vi "Modbus Master.vi"() -> ()   [LabVIEW 2021]
uses:
  TypeDefs/Tester Object.ctl
  TypeDefs/UIControlReferences.ctl
  TypeDefs/Devices Cluster.ctl
  Modbus/Modbus Cluster.ctl
  <vilib>/NI/Modbus Library/API/Master/Modbus Master.lvclass
  Modbus/Modbus Address Cluster.ctl
  <vilib>/NI/Modbus Library/API/Slave/Modbus Slave.lvclass
  DAQ/DAQNav/DAQNav Cluster.ctl
  DAQ/DAQNav/Analog Cluster.ctl
panel:
  out "Register Values":dbl[](array[numeric])
  in  "stop":bool
  out "error out":errorcluster
  out "Motor Speed":dbl
  out "Temperature":dbl
  out "Positioning":dbl
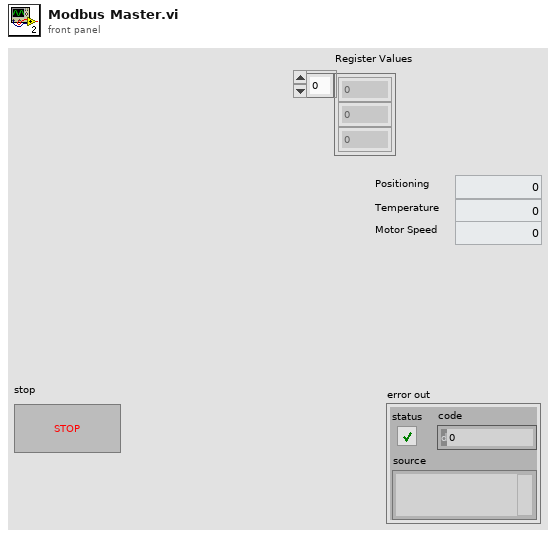
[diagram p1: front panel]
types:
  T1 = typedef "Tester Object.ctl" = cluster{"Program Properties":cluster{"Application Path":path}, "Control Refnum":T2, "Devices":T3}
  T2 = typedef "UIControlReferences.ctl" = cluster{"Tree Refnum ":refnum<vi>, "Graph1 Refnum":refnum<vi>, "Graph2 Refnum":refnum<vi>, "Temperature Refnum":refnum<vi>, "Sensor Str Refnum":refnum<vi>, "Motor Speed Refnum":refnum<vi>, "Equipment Connected Refnum":refnum<vi>, "Calibrated Refnum":refnum<vi>, "Positioning Refnum":refnum<vi>, "Servo On Refnum":refnum<vi>, "seqPauseButton":refnum<vi>, "seqStartButton":refnum<vi>, "seqStopButton":refnum<vi>}
  T3 = typedef "Devices Cluster.ctl" = cluster{"Modbus":T4, "TCP/IP":cluster{"connection ID":refnum<k5>, "Address":string}, "DAQ Device":T6}
  T4 = typedef "Modbus Cluster.ctl" = cluster{"Modbus master instance":refnum<class "Modbus Master.lvclass">, "MB Holding Register":T5[], "MB Coils":T5[], "TCP slave instance":refnum<class "Modbus Slave.lvclass">}
  T5 = typedef "Modbus Address Cluster.ctl" = cluster{"Session":string, "Device Type":string, "Memory Block":string, "Function":string, "Address":u16}
  T6 = typedef "DAQNav Cluster.ctl" = cluster{"AI task out":i32, "AI Found?":bool, "AO task out":i32, "AO Found?":bool, "Analog Input List":T7[], "Analog Out List":T7[]}
  T7 = typedef "Analog Cluster.ctl" = cluster{"Name":string, "Device Type":string, "Channel":i32}
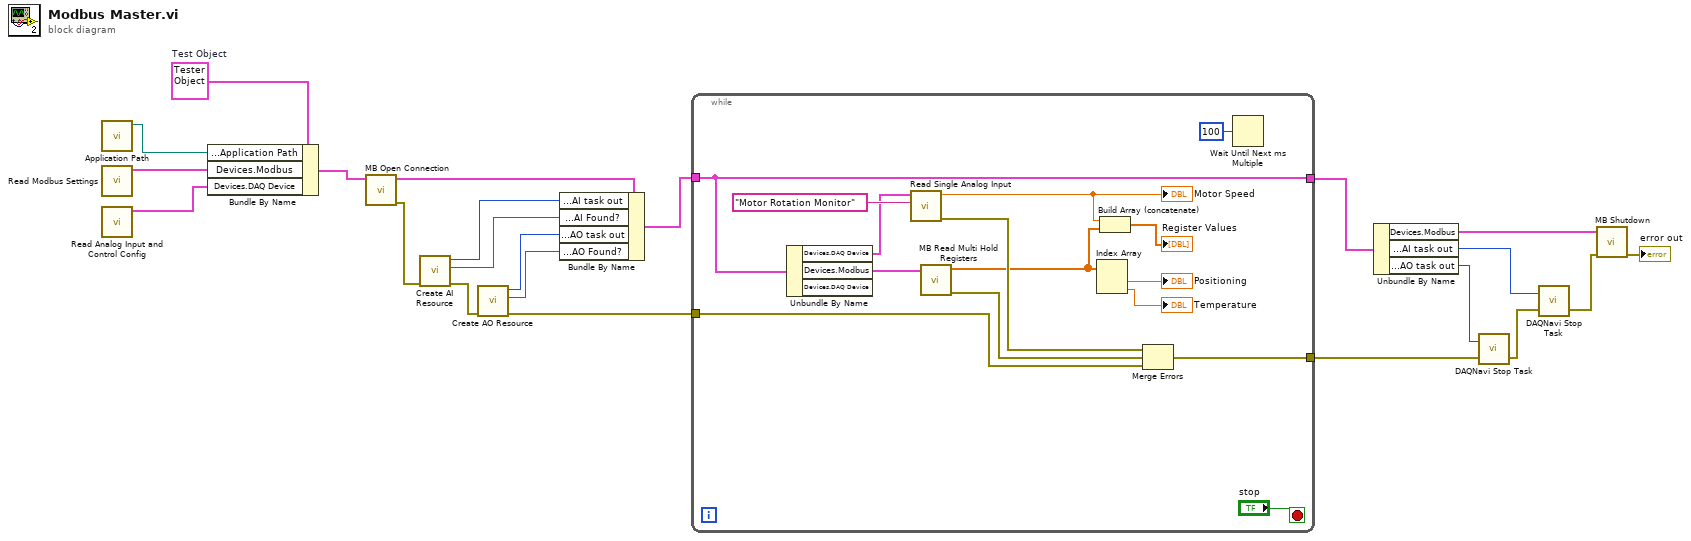
[diagram p0: block diagram]
diagram:
  w22 = T1 {"Program Properties"={"Application Path"=path ""}, "Control Refnum"={"Tree Refnum "=refnum, "Graph1 Refnum"=refnum, "Graph2 Refnum"=refnum, "Temperature Refnum"=refnum, "Sensor Str Refnum"=refnum, "Motor Speed Refnum"=refnum, "Equipment Connected Refnum"=refnum, "Calibrated Refnum"=refnum, "Positioning Refnum"=refnum, "Servo On Refnum"=refnum, "seqPauseButton"=refnum, "seqStartButton"=refnum, "seqStopButton"=refnum}, "Devices"={"Modbus"={"Modbus master instance"=refnum, "MB Holding Register"=[], "MB Coils"=[], "TCP slave instance"=refnum}, "TCP/IP"={"connection ID"=refnum, "Address"=""}, "DAQ Device"={"AI task out"=0, "AI Found?"=FALSE, "AO task out"=0, "AO Found?"=FALSE, "Analog Input List"=[], "Analog Out List"=[]}}}  # Test Object
  n1 = call "Application Path.vi"() -> ("appended path"=w1:path)  [unwired: 11 in]
  n2 = call "Read Modbus Settings.vi"() -> ("Devices.Modbus"=w21:T4)  [unwired: 11 in]
  n3 = call "Read Analog Input and Control Config.vi"() -> ("daq cluster"=w20:T6)  [unwired: 11 in]
  n4 = Bundle By Name(cluster=w22, "Program Properties.Application Path"=w1, "Devices.Modbus"=w21, "Devices.DAQ Device"=w20) -> (w19:T1)
  n5 = call "MB Open Connection.vi"("Test Object in"=w19) -> ("error out"=w3:errorcluster, "Test Object out"=w18:T1)  [unwired: 9 in]
  n6 = call "Create AI Resource.vi"("error in (no error)"=w3) -> ("error out"=w2:errorcluster, "found?"=w16:bool, "task out"=w17:i32)  [unwired: 8 in]
  n7 = call "Create AO Resource.vi"("error in (no error)"=w2) -> ("error out"=w4:errorcluster, "found?"=w14:bool, "task out"=w15:i32)  [unwired: 8 in]
  n8 = Bundle By Name(cluster=w18, "Devices.DAQ Device.AI task out"=w17, "Devices.DAQ Device.AI Found?"=w16, "Devices.DAQ Device.AO task out"=w15, "Devices.DAQ Device.AO Found?"=w14) -> (w13:T1)
  n9 = while {
    tunnel: w13 -> [w34]
    tunnel: [w34] -> w9
    tunnel: [w33] -> w8
    tunnel: w4 -> [w32]
    stop <- "stop" stop-if-true
    n10 = Unbundle By Name(w34) -> ("Devices.DAQ Device"=w23:T6, "Devices.Modbus"=w37:T4)  [unwired: 1 out]
    n11 = call "Read Single Analog Input.vi"("Parameter Name"="Motor Rotation Monitor", "Devices.DAQ Device"=w23) -> ("error out"=w28:errorcluster, "data"=w26:dbl)  [unwired: 7 in, 1 out]
    "Motor Speed" <- w26
    n12 = call "MB Read Multi Hold Registers.vi"("Devices.Modbus"=w37) -> ("error out"=w27:errorcluster, "Register Values"=w25:dbl[])  [unwired: 9 in]
    n13 = Index Array(array=w25) -> (element #1=→"Positioning":dbl, element #2=→"Temperature":dbl)  [unwired: 2 in]
    n14 = Build Array (concatenate)(w26, w25) -> (→"Register Values":dbl[])
    n15 = Merge Errors(w28, w27, w32) -> (w33:errorcluster)
    n16 = Wait Until Next ms Multiple(millisecond multiple=u32 100) -> ()  [unwired: 1 out]
  }
  n17 = Unbundle By Name(w9) -> ("Devices.Modbus"=w12:T4, "Devices.DAQ Device.AI task out"=w11:i32, "Devices.DAQ Device.AO task out"=w10:i32)
  n18 = call <userlib>:"DAQNavi Stop Task.vi"("error in (no error)"=w8, "task in"=w10) -> ("error out"=w7:errorcluster)  [unwired: 1 out]
  n19 = call <userlib>:"DAQNavi Stop Task.vi"("error in (no error)"=w7, "task in"=w11) -> ("error out"=w6:errorcluster)  [unwired: 1 out]
  n20 = call "MB Shutdown.vi"("error in (no error)"=w6, "Devices"=w12) -> ("error out"=→"error out":errorcluster)  [unwired: 9 in]
